vi "SeqEditor_StepMLSTpaste.vi"(8 "error in (no error)":errorcluster, 11 "NLTest in":refnum<class "NLTest.lvclass">) -> (0 "error out":errorcluster, 3 "NLTest out":refnum<class "NLTest.lvclass">)   [LabVIEW 2017, in "NLTest.lvclass"]
uses:
  NLTest.lvclass
  NLTest.lvclass/NLTest.ctl
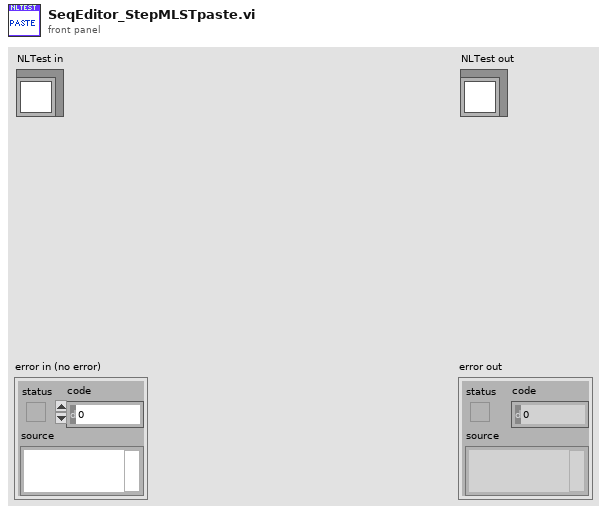
[diagram p1: front panel]
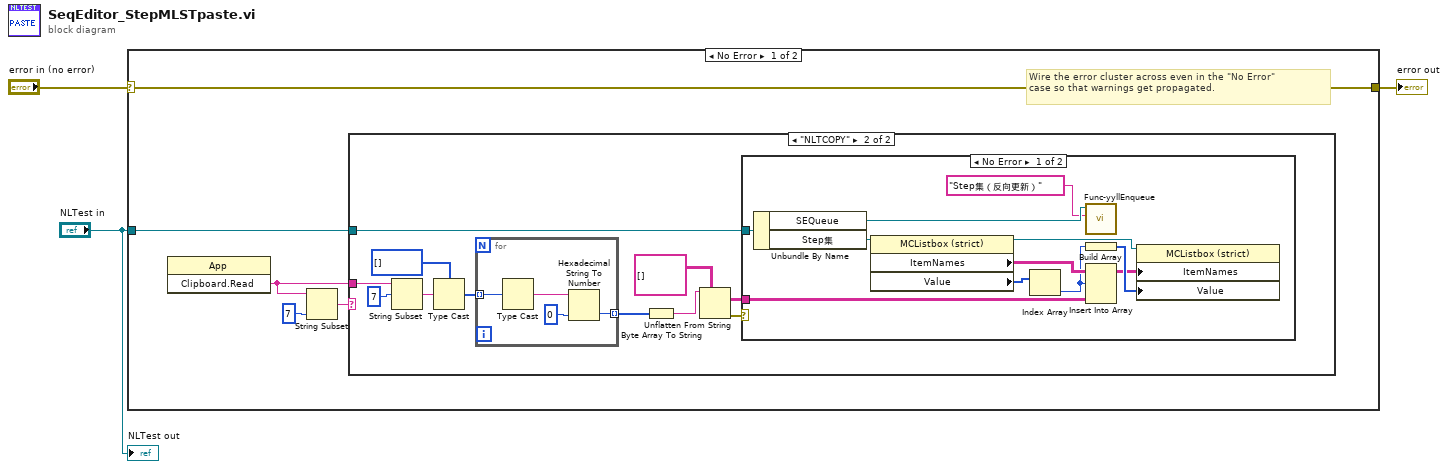
[diagram p0: block diagram]
diagram:
  n1 = case shown="No Error" "error in (no error)" {
    selector: "error in (no error)" -> [w8 w35]
    tunnel: [w8 w35] -> w2
    tunnel: "NLTest in" -> [w4 _]
    frame No Error {
      # "Wire the error cluster across even in the \"No Error\"\ncase so that warnings get propagated."
      n2 = invoke class="App" method="Clipboard.Read"() -> ("Read Clipbrd"=w5:string)  [unwired: 3 in, 2 out]
      n3 = String Subset(string=w5, length (rest)=7 ("offset (0)")) -> (substring=w6:string)  [unwired: 1 in]
      n4 = case shown="\"NLTCOPY\"" w6 {
        tunnel: w5 -> [_ w19]
        tunnel: w4 -> [_ w9]
        frame "False", Default {
        }
        frame "NLTCOPY" {
          n5 = String Subset(string=w19, offset (0)=7) -> (substring=w14:string)  [unwired: 1 in]
          n6 = Type Cast(type=u16[] [], x=w14) -> (*(type *) &x=w16:u16[])
          n7 = for {
            tunnel: w16 -> [w34] mode=indexing
            tunnel: [w31] -> w15 mode=indexing
            n8 = Type Cast(x=w34) -> (*(type *) &x=w33:string)  [unwired: 1 in]
            n9 = Hexadecimal String To Number(string=w33, default (0uL)=u8 0 ("default (0 U32)")) -> (number=w31:u8)  [unwired: 1 in, 1 out]
          }
          n10 = Byte Array To String(unsigned byte array=w15) -> (string=w13:string)
          n11 = Unflatten From String(type=string[][] [] ("ItemNames"), binary string=w13) -> (value=w10:string[][], error out=w11:errorcluster)  [unwired: 3 in, 1 out]
          n12 = case shown="No Error" w11 {
            tunnel: w10 -> [w24 _]
            tunnel: w9 -> [w30 _]
            frame No Error {
              n13 = Unbundle By Name(w30) -> ("SEQueue"=w29:refnum<queue>, "Step集"=w27:refnum<vi>)
              n14 = property class="MCListbox (strict)"(reference=w27) -> (reference out=w20:refnum<vi>, "ItemNames"=w25:string[][], "Value"=w26:i32[])  [unwired: 1 in, 1 out]
              n15 = Index Array(array=w26) -> (element=w23:i32)  [unwired: 1 in]
              n16 = call "Func-yyllEnqueue.vi"("cmd"="Step集（反向更新）", "queue in"=w29) -> ()  [unwired: 7 in, 3 out]
              n17 = Build Array(w23) -> (w22:i32[])
              n18 = Insert Into Array(array=w25, index (row)=w23, new element=w24) -> (w21:string[][])  [unwired: 1 in]
              n19 = property class="MCListbox (strict)"(reference=w20, "ItemNames"=w21, "Value"=w22) -> ()  [unwired: 1 in, 2 out]
            }
            frame Error {
            }
          }
        }
      }
    }
    frame Error {
    }
  }
  "error out" <- w2
  "NLTest out" <- "NLTest in"
